vi "Move Prices.vi"(11 "market":T1) -> (3 "market out":T1)   [LabVIEW 2020, in "Full Featured MCP Server.lvlib"]
doc: "Moves every price by one second and appends it to the price history. The return of each stock comes from Price Return.vi: trend, momentum left by news, the move of the whole market and of the sector, random noise and the shock of this second. Afterwards the shock is used up and momentum and nervousness fade a little."
uses:
  Full Featured MCP Server.lvlib
  Market State.ctl
  News Item.ctl
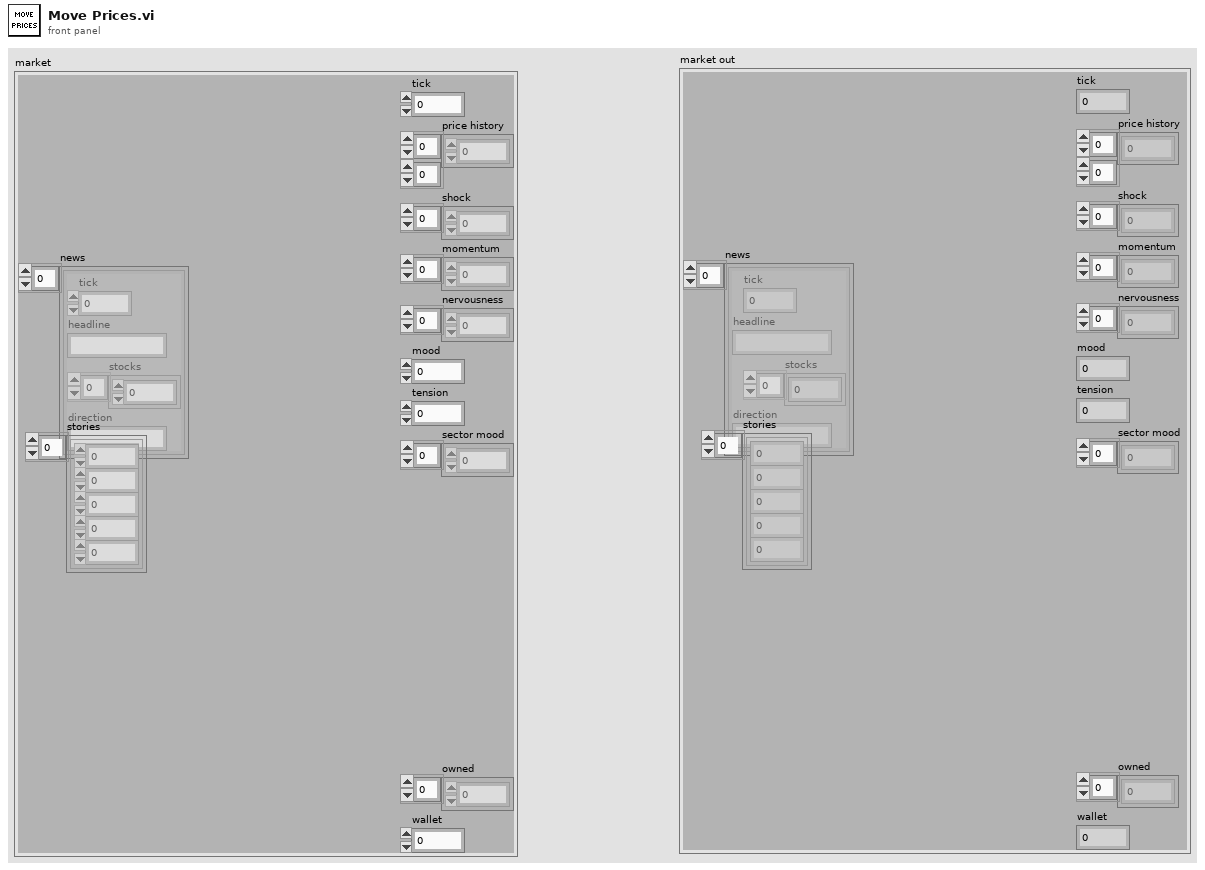
[diagram p1: front panel]
types:
  T1 = typedef "Full Featured MCP Server.lvlib/Market State.ctl" = cluster{"tick":i32, "price history":dbl[][], "shock":dbl[], "momentum":dbl[], "nervousness":dbl[], "mood":dbl, "tension":dbl, "sector mood":dbl[], "news":T2[], "stories":cluster{"arc":i32, "step":i32, "due":i32, "stock":i32, "other":i32}[], "owned":i32[], "wallet":dbl}
  T2 = typedef "Full Featured MCP Server.lvlib/News Item.ctl" = cluster{"tick":i32, "headline":string, "stocks":i32[], "direction":string}
  T3 = cluster{"name":string, "sector":i32, "quality":i32, "start price":dbl, "drift":dbl, "volatility":dbl, "beta":dbl, "jumpiness":dbl, "description":string}[]
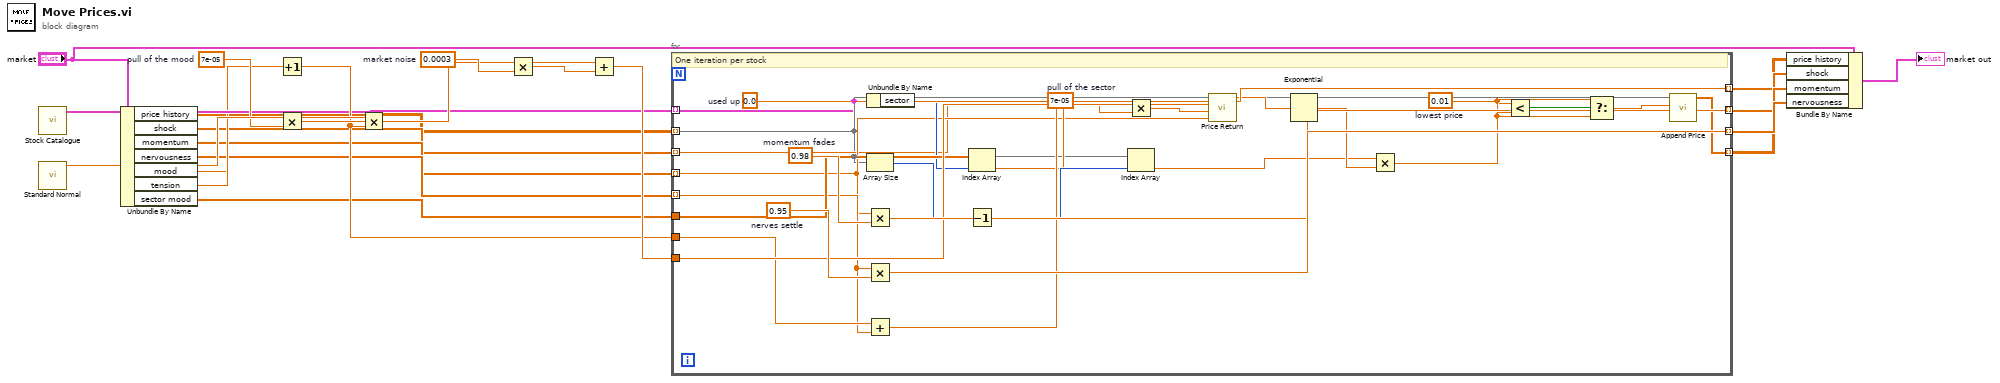
[diagram p0: block diagram]
diagram:
  w15 = 0.0003  # market noise
  w11 = 7e-05  # pull of the mood
  n1 = call "Stock Catalogue.vi"() -> ("stocks"=w9:T3)  [unwired: 10 in, 1 out]
  n2 = call "Standard Normal.vi"() -> ("number"=w13:dbl)  [unwired: 11 in]
  n3 = Unbundle By Name("market") -> ("price history"=w2:dbl[][], "shock"=w3:dbl[], "momentum"=w4:dbl[], "nervousness"=w5:dbl[], "mood"=w6:dbl, "tension"=w7:dbl, "sector mood"=w8:dbl[])
  n4 = Increment(x=w7) -> (x+1=w10:dbl)
  n5 = Multiply(x=w6, y=w11) -> (x*y=w12:dbl)
  n6 = Multiply(x=w13, y=w10) -> (x*y=w14:dbl)
  n7 = Multiply(x=w14, y=w15) -> (x*y=w16:dbl)
  n8 = Add(x=w12, y=w16) -> (x+y=w17:dbl)
  n9 = for {
    tunnel: [w46] -> w19 mode=indexing
    tunnel: w9 -> [w23] mode=indexing
    tunnel: w2 -> [w24] mode=indexing
    tunnel: w3 -> [w25] mode=indexing
    tunnel: w4 -> [w26] mode=indexing
    tunnel: w5 -> [w27] mode=indexing
    tunnel: w8 -> [w29]
    tunnel: w10 -> [w33]
    tunnel: [w48] -> w20 mode=indexing
    tunnel: [w50] -> w21 mode=indexing
    tunnel: w17 -> [w35]
    tunnel: [w45] -> w18 mode=indexing
    w49 = 0.95  # nerves settle
    w47 = 0.98  # momentum fades
    w46 = 0.0  # used up
    w42 = 0.01  # lowest price
    w31 = 7e-05  # pull of the sector
    # "One iteration per stock"
    n10 = Unbundle By Name(w23) -> ("sector"=w28:i32)
    n11 = Array Size(array=w24) -> (size(s)=w37:i32)
    n12 = Multiply(x=w26, y=w47) -> (x*y=w48:dbl)
    n13 = Multiply(x=w27, y=w49) -> (x*y=w50:dbl)
    n14 = Add(x=w33, y=w27) -> (x+y=w34:dbl)
    n15 = Index Array(array=w29, index=w28) -> (element=w30:dbl)
    n16 = Decrement(x=w37) -> (x-1=w38:i32)
    n17 = Multiply(x=w30, y=w31) -> (x*y=w32:dbl)
    n18 = Index Array(array=w24, index=w38) -> (element=w39:dbl)
    n19 = call "Price Return.vi"("nervousness"=w34, "shock"=w25, "momentum"=w26, "sector move"=w32, "market move"=w35, "stock"=w23) -> ("return"=w36:dbl)  [unwired: 5 in]
    n20 = Exponential(1:w36) -> (0:w40:dbl)
    n21 = Multiply(x=w39, y=w40) -> (x*y=w41:dbl)
    n22 = Less?(x=w41, y=w42) -> (x < y?=w43:bool)
    n23 = Select(t=w42, s=w43, f=w41) -> (s? t:f=w44:dbl)
    n24 = call "Append Price.vi"("new price"=w44, "prices"=w24) -> ("prices out"=w45:dbl[])  [unwired: 9 in]
  }
  n25 = Bundle By Name(cluster="market", "price history"=w18, "shock"=w19, "momentum"=w20, "nervousness"=w21) -> (→"market out":T1)
